vi "Stop Task.vi"(8 "error in (no error)":errorcluster caption="错误输入（无错误）", 11 "nRunMode":i32) -> (0 "error out":errorcluster caption="错误输出", 3 "function return":i32)   [LabVIEW 2017, in "smncsftmt.lvlib"]
doc: "__declspec(dllexport) int StopTask(int nRunMode);"
uses:
  smncsftmt.lvlib
  smncsftmt.dll
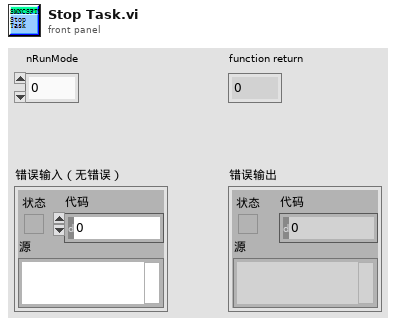
[diagram p1: front panel]
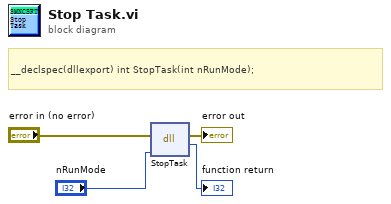
[diagram p0: block diagram]
diagram:
  # "__declspec(dllexport) int StopTask(int nRunMode);"
  n1 = dll-call lib="PTH2oabs CUsersaDesktop\nLABVIEW范例National InstrumentsLabVIEW 2017user.lib\tsmncsftmtsmncsftmt.*" fn="StopTask"(error in="error in (no error)", "nRunMode"="nRunMode") -> (error out=→"error out":errorcluster, →"function return":i32)  [unwired: 3 in, 1 out]
